vi "DSS-Tests-error_message.vi"(8 "error in":errorcluster, 9 "prefix":string, 10 "message in":string, 11 "pass in":bool) -> (0 "error out":errorcluster, 2 "message":string, 3 "pass":bool)   [LabVIEW 2020, in "DSS-Tests.lvlib"]
doc: "Turns a check result into an assertion result: pass only without an error, the message replaced by the error code and source when there is one, and prefixed with the case name."
uses:
  DSS-Tests.lvlib
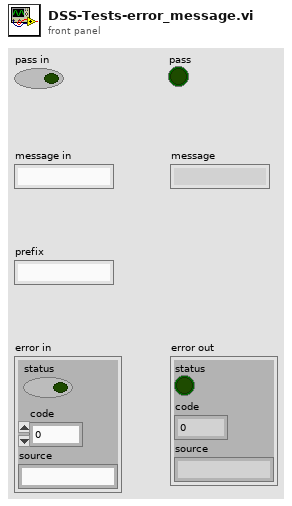
[diagram p1: front panel]
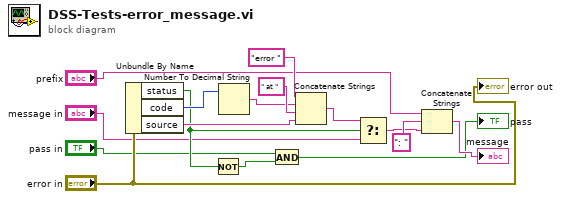
[diagram p0: block diagram]
diagram:
  n1 = Unbundle By Name("error in") -> ("status"=w5:bool, "code"=w6:i32, "source"=w7:string)
  n2 = Not(x=w5) -> (.not. x?=w8:bool)
  n3 = Number To Decimal String(number=w6) -> (decimal integer string=w10:string)  [unwired: 1 in]
  n4 = And(x="pass in", y=w8) -> (x .and. y?=→"pass":bool)
  n5 = Concatenate Strings("error " ("t error"), w10, " at " ("t at"), w7) -> (w13:string)
  n6 = Select(t=w13, s=w5, f="message in") -> (s? t:f=w14:string)
  n7 = Concatenate Strings("prefix", ": " ("t sep"), w14) -> (→"message":string)
  "error out" <- "error in"
